vi "Scan Engine Main Page.vi"(8 "error in (no error)":errorcluster, 11 "Node Ptr":T1 format="%.0x") -> (0 "error out":errorcluster)   [LabVIEW 2020, in "SEECD System Explorer.lvlib"]
uses:
  SEECD System Explorer.lvlib
  <vilib>/NI VeriStand/Custom Device API/Custom Device Item Ref.ctl
  <vilib>/NI VeriStand/Custom Device API/Custom Device API.lvlib
  Scripting/Scan Engine Scripting.lvlib
panel:
  in  "disable refresh modules":bool
  in  "Delay after FPGA load (s)":u16
  in  "SHDocVw.IWebBrowser2":refnum<k7>(container)
  in  "Scan Engine Decimation":u16=1 min=1 max=100
  in  "Sync to Scan?":bool
  in  "Header":cluster{"Section Name":string}={"Section Name"="Scan Engine and EtherCAT Custom Device Settings"}
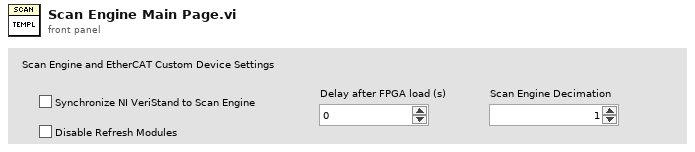
[diagram p1: front panel]
types:
  T1 = typedef "Custom Device API.lvlib/Custom Device Item Ref.ctl" = u64
  T2 = typedef "Custom Device API.lvlib/Custom Device Commands.ctl" = enum16{"Default", "Item renamed", "Shutdown", "Dynamic button pressed"}
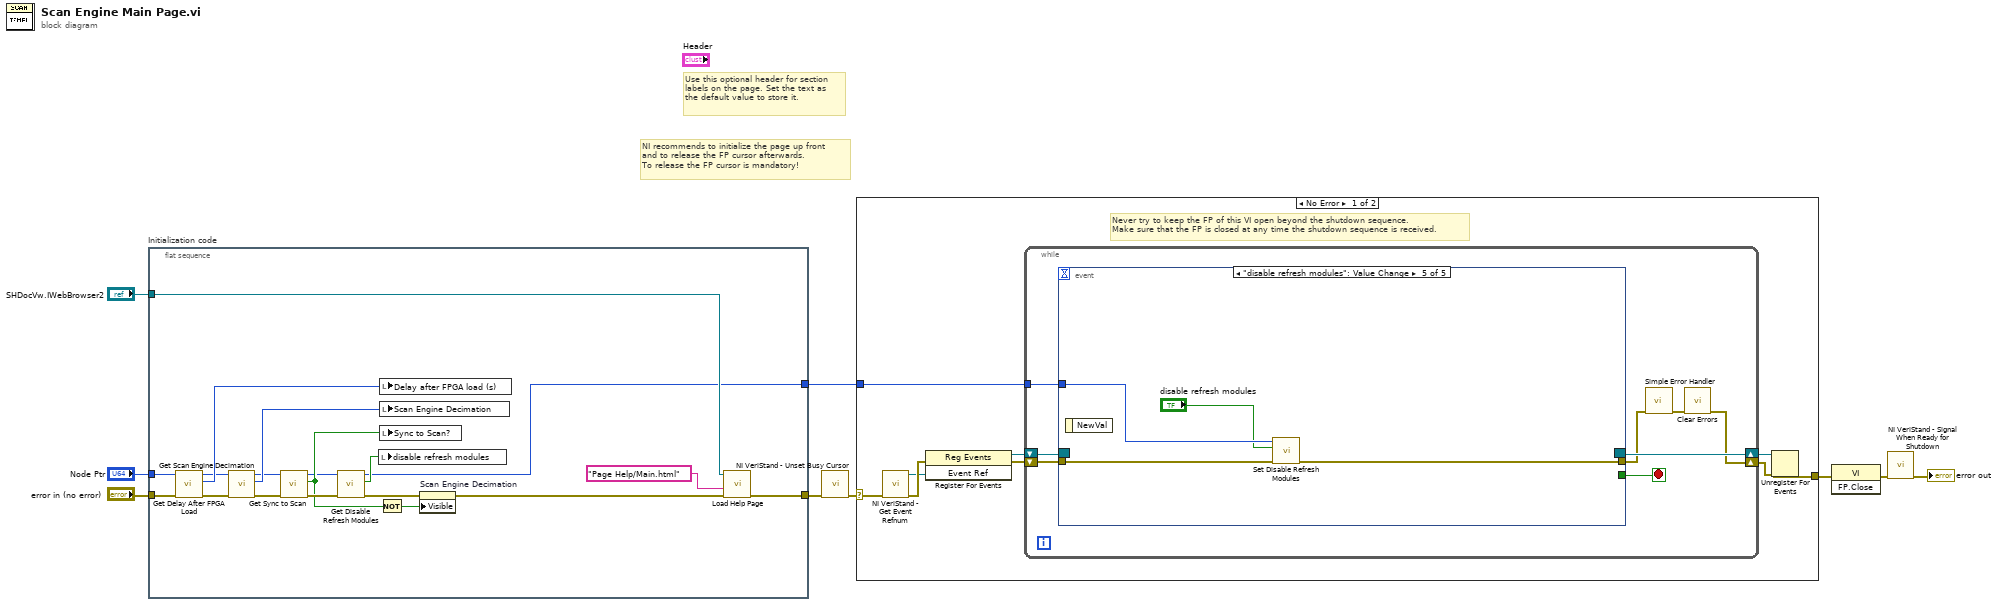
[diagram p0: block diagram]
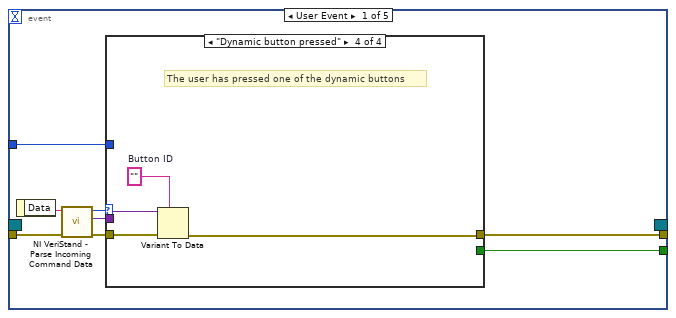
[diagram p2: hidden frame]
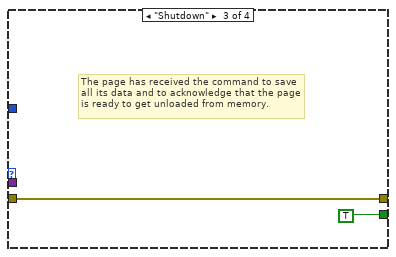
[diagram p5: hidden frame]
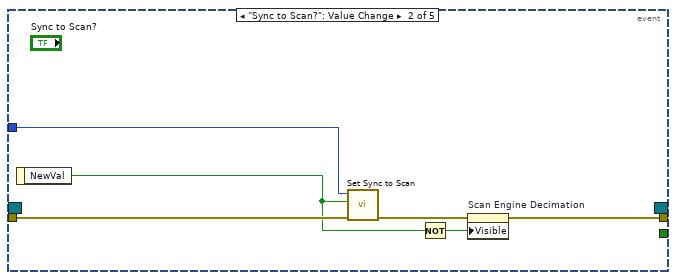
[diagram p6: hidden frame]
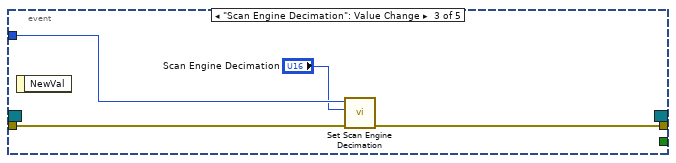
[diagram p7: hidden frame]
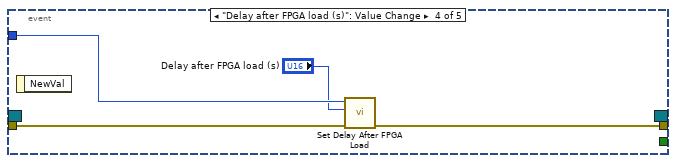
[diagram p8: hidden frame]
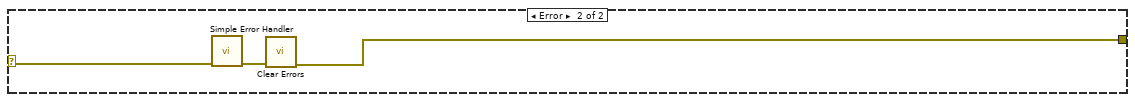
[diagram p9: hidden frame]
diagram:
  # "Use this optional header for section labels on the page. Set the text as the default value to store it."
  # "NI recommends to initialize the page up front\nand to release the FP cursor afterwards.\nTo release the FP cursor is mandatory!"
  n1 = flat-sequence "Initialization code" {
    tunnel: "error in (no error)" -> [w26]
    tunnel: "Node Ptr" -> [w27]
    tunnel: [w16] -> w5
    tunnel: [w10] -> w2
    tunnel: "SHDocVw.IWebBrowser2" -> [w15]
    frame #0 {
      n2 = call "Get Delay After FPGA Load.vi"("error in"=w26, "scan engine custom device ref in"=w27) -> ("error out"=w23:errorcluster, "delay after FPGA load (s)"=w25:u16, "scan engine custom device ref out"=w24:T1)  [unwired: 7 in]
      n3 = call "Get Scan Engine Decimation.vi"("error in"=w23, "scan engine custom device ref in"=w24) -> ("error out"=w20:errorcluster, "scan engine decimation"=w22:u16, "scan engine custom device ref out"=w21:T1)  [unwired: 7 in]
      n4 = call "Get Sync to Scan.vi"("error in"=w20, "scan engine custom device ref in"=w21) -> ("error out"=w19:errorcluster, "sync to scan"=w18:bool, "scan engine custom device ref out"=w12:T1)  [unwired: 7 in]
      n5 = call "Get Disable Refresh Modules.vi"("error in"=w19, "scan engine custom device ref in"=w12) -> ("error out"=w13:errorcluster, "disable refresh modules"=w11:bool, "scan engine custom device ref out"=w10:T1)  [unwired: 7 in]
      n6 = local write "disable refresh modules"(w11) -> ()
      n7 = Not(x=w18) -> (.not. x?=w28:bool)
      n8 = local write "Delay after FPGA load (s)"(w25) -> ()
      n9 = local write "Scan Engine Decimation"(w22) -> ()
      n10 = local write "Sync to Scan?"(w18) -> ()
      n11 = property on="Scan Engine Decimation" class="DigNum (strict)"(error in=w13, "Visible"=w28) -> (error out=w17:errorcluster)  [unwired: 1 in, 1 out]
      n12 = call "Load Help Page.vi"("error in (no error)"=w17, "HTML File to Load"="Page Help/Main.html" ("name or relative path"), "Browser"=w15) -> ("error out"=w16:errorcluster)  [unwired: 8 in]
    }
  }
  n13 = call <vilib>:"NI VeriStand - Unset Busy Cursor.vi"("error in (no error)"=w5) -> ("error out"=w4:errorcluster)  [unwired: 10 out]
  n14 = case shown="No Error" w4 {
    selector: w4 -> [w29 w82]
    tunnel: [w34 w80] -> w9
    tunnel: w2 -> [w30 _]
    frame No Error {
      # "Never try to keep the FP of this VI open beyond the shutdown sequence.\nMake sure that the FP is closed at any time the shutdown sequence is received."
      n15 = call <vilib>:"NI VeriStand - Get Event Refnum.vi"("error in (no error)"=w29) -> ("error out"=w37:errorcluster, "Event Ref"=w33:refnum<user-event>)  [unwired: 9 out]
      n16 = register-events(error in=w37, w33) -> (reference out=w31:refnum<event-registration>, error out=w32:errorcluster)  [unwired: 1 in]
      n17 = while {
        tunnel: w30 -> [w41]
        shift-right: [w38] -> w35
        shift-left: w32 -> [w44]
        shift-right: [w45] -> w36
        shift-left: w31 -> [w43]
        stop <- w42 stop-if-true
        n18 = event shown="[4] \"disable refresh modules\": Value Change" {
          selector: w43 -> [_ _ _ _ _]
          dyn-events: [_ _ _ _ _] -> w45
          timeout: _ -> [_ _ _ _ _]
          tunnel: w44 -> [w53 w66 w71 w75 w79]
          tunnel: [w49 _ _ _ _] -> w42
          tunnel: [w48 w63 w70 w74 w76] -> w40
          tunnel: w41 -> [w47 w67 w69 w73 w78]
          event User Event {
            n19 = event-data() -> ("Data"=w52:string)  [unwired: 1 out]
            n20 = call <vilib>:"NI VeriStand - Parse Incoming Command Data.vi"("error in (no error)"=w53, "Incoming data"=w52) -> ("error out"=w51:errorcluster, "Outgoing data"=w46:variant, "Action"=w50:T2)  [unwired: 7 out]
            n21 = case shown="\"Dynamic button pressed\"" w50 {
              tunnel: w51 -> [w54 w55 w56 w61]
              tunnel: [_ _ TRUE _] -> w49
              tunnel: [w54 w55 w56 w58] -> w48
              tunnel: w47 -> [_ _ _ _]
              tunnel: w46 -> [_ _ _ w60]
              frame "Default", Default {
              }
              frame "Item renamed" {
              }
              frame "Shutdown" {
                # "The page has received the command to save all its data and to acknowledge that the page is ready to get unloaded from memory."
              }
              frame "Dynamic button pressed" {
                w59 = ""  # Button ID
                # "The user has pressed one of the dynamic buttons"
                n22 = Variant To Data(error in=w61, type=w59, Variant=w60) -> (error out=w58:errorcluster)  [unwired: 1 out]
              }
            }
          }
          event "Sync to Scan?": Value Change {
            n23 = event-data() -> ("NewVal"=w62:bool)  [unwired: 1 out]
            n24 = call "Set Sync to Scan.vi"("error in"=w66, "sync to scan"=w62, "scan engine custom device ref in"=w67) -> ("error out"=w64:errorcluster)  [unwired: 7 in, 1 out]
            n25 = Not(x=w62) -> (.not. x?=w65:bool)
            n26 = property on="Scan Engine Decimation" class="DigNum (strict)"(error in=w64, "Visible"=w65) -> (error out=w63:errorcluster)  [unwired: 1 in, 1 out]
          }
          event "Scan Engine Decimation": Value Change {
            n27 = event-data() -> ()  [unwired: 2 out]
            n28 = call "Set Scan Engine Decimation.vi"("error in"=w71, "scan engine decimation"="Scan Engine Decimation", "scan engine custom device ref in"=w69) -> ("error out"=w70:errorcluster)  [unwired: 7 in, 1 out]
          }
          event "Delay after FPGA load (s)": Value Change {
            n29 = event-data() -> ()  [unwired: 2 out]
            n30 = call "Set Delay After FPGA Load.vi"("error in"=w75, "delay after FPGA load (s)"="Delay after FPGA load (s)", "scan engine custom device ref in"=w73) -> ("error out"=w74:errorcluster)  [unwired: 7 in, 1 out]
          }
          event "disable refresh modules": Value Change {
            n31 = event-data() -> ()  [unwired: 2 out]
            n32 = call "Set Disable Refresh Modules.vi"("error in"=w79, "disable refresh modules"="disable refresh modules", "scan engine custom device ref in"=w78) -> ("error out"=w76:errorcluster)  [unwired: 7 in, 1 out]
          }
        }
        n33 = call <vilib>:"Simple Error Handler.vi"("error in (no error)"=w40) -> ("error out"=w39:errorcluster)  [unwired: 1 in, 7 out]
        n34 = call <vilib>:"Clear Errors.vi"("error in (no error)"=w39) -> ("error out"=w38:errorcluster)  [unwired: 1 in, 5 out]
      }
      n35 = Unregister For Events(event registration refnum=w36, error in=w35) -> (error out=w34:errorcluster)
    }
    frame Error {
      n36 = call <vilib>:"Simple Error Handler.vi"("error in (no error)"=w82) -> ("error out"=w81:errorcluster)  [unwired: 1 in, 7 out]
      n37 = call <vilib>:"Clear Errors.vi"("error in (no error)"=w81) -> ("error out"=w80:errorcluster)  [unwired: 1 in, 5 out]
    }
  }
  n38 = invoke class="VI" method="FP.Close"(error in=w9) -> (error out=w8:errorcluster)  [unwired: 2 in, 2 out]
  n39 = call <vilib>:"NI VeriStand - Signal When Ready for Shutdown.vi"("error in (no error)"=w8) -> ("error out"=→"error out":errorcluster)  [unwired: 10 out]
